vi "PicoScope6000aAWG.vi"(0 "Handle In":i16=16384, 1 "General AWG Settings":T4={"Peak-to-Peak Voltage"=2.0, "Offset Voltage"=0.0, "Wave Type"=17, "Sweep Type"=0, "Cycles"=10, "Trigger Type"=0, "Trigger Source"=4, "sigGenEnabled"=TRUE, "Trigger Enabled"=FALSE, "autoTriggerPicoSeconds"=0} {"Trigger Source" items=["None"=0, "Scope Trigger"=1, "Software Trigger"=4, "Trigger Raw"=5]; "Trigger Type" items=["Rising", "Falling", "Gate High", "Gate Low"]; "Sweep Type" items=["Up", "Down", "Up-Down", "Down-Up"]; "Wave Type" items=["Sine"=17, "Square"=18, "Triangle"=19, "Ramp Up"=20, "Ramp Down"=21, "Sinc"=22, "Gaussian"=23, "Half Sine"=24, "DC"=1024, "PWM"=4096, "White Noise"=8193, "PRBS"=8194, "Arbitrary"=268435456]; "Offset Voltage" format="%#_6p"; "Peak-to-Peak Voltage" format="%#_6p"}, 2 "Standard Waveform Settings":T3={"(Start) Frequency"=1000.0, "Stop Frequency"=5000.0, "Increment"=1.0, "Dwell Time (seconds)"=0.001, "Sweep Enabled"=FALSE} {"Dwell Time (seconds)" format="%#_6p"; "Stop Frequency" min=0.03 max=1000000.0 format="%#_6p"; "(Start) Frequency" min=0.03 max=1000000.0 format="%#_6p"}, 3 "Arbitrary Waveform Settings":T2 {"Index Mode" items=["Single", "Dual", "Quad"]}, 11 "error in":errorcluster, 12 "Duty Cycle":T1={"Use Duty Cycle"=FALSE, "dutyCyclePercent"=20.0}) -> (4 "Handle Out":i16=16384, 13 "Trigger Source Out":u32=4, 14 "Arbitrary\nWaveform Graph":i16[](graph), 15 "error out":errorcluster)   [LabVIEW 2010]
doc: "This VI can be used to control the arbitrary waveform generator. Standard waveforms can be selected or arbitrary waveform can be selected under 'Wave Type'. There are three settings clusters: general settings that apply to both arbitrary and standard waveforms, settings that apply only to standard waveforms and settings that apply only to arbitrary waveforms. It is not necessary to connect all of these clusters if only using arbitrary waveforms or only using standard waveforms are required.\n\nWhen selecting arbitrary waveform, it is necessary to specify a text file containing the wave form. This text file should have a single value on each line in the range -1 to 1. For further information on the settings, see descriptions of ps3000aSetSigGenBuiltIn and ps3000aSetSigGenArbitrary."
uses:
  ps6000a.dll
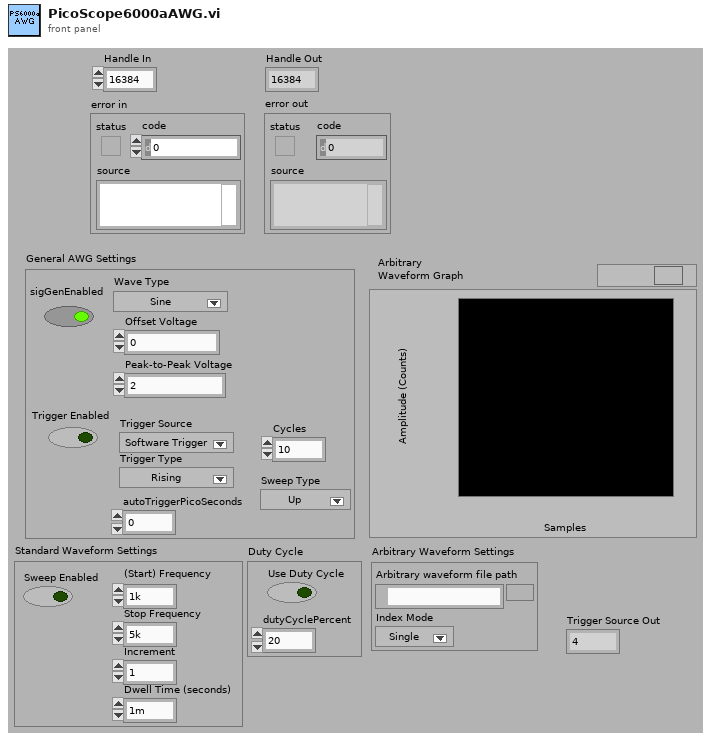
[diagram p1: front panel]
types:
  T1 = cluster{"Use Duty Cycle":bool, "dutyCyclePercent":dbl}
  T2 = cluster{"Arbirary waveform file path":path, "Index Mode":u32}
  T3 = cluster{"(Start) Frequency":dbl, "Stop Frequency":dbl, "Increment":dbl, "Dwell Time (seconds)":dbl, "Sweep Enabled":bool}
  T4 = cluster{"Peak-to-Peak Voltage":dbl, "Offset Voltage":dbl, "Wave Type":u32, "Sweep Type":u32, "Cycles":u64, "Trigger Type":u32, "Trigger Source":u32, "sigGenEnabled":bool, "Trigger Enabled":bool, "autoTriggerPicoSeconds":u64}
  T5 = cluster{"status":bool, "code":u32, "source":string}
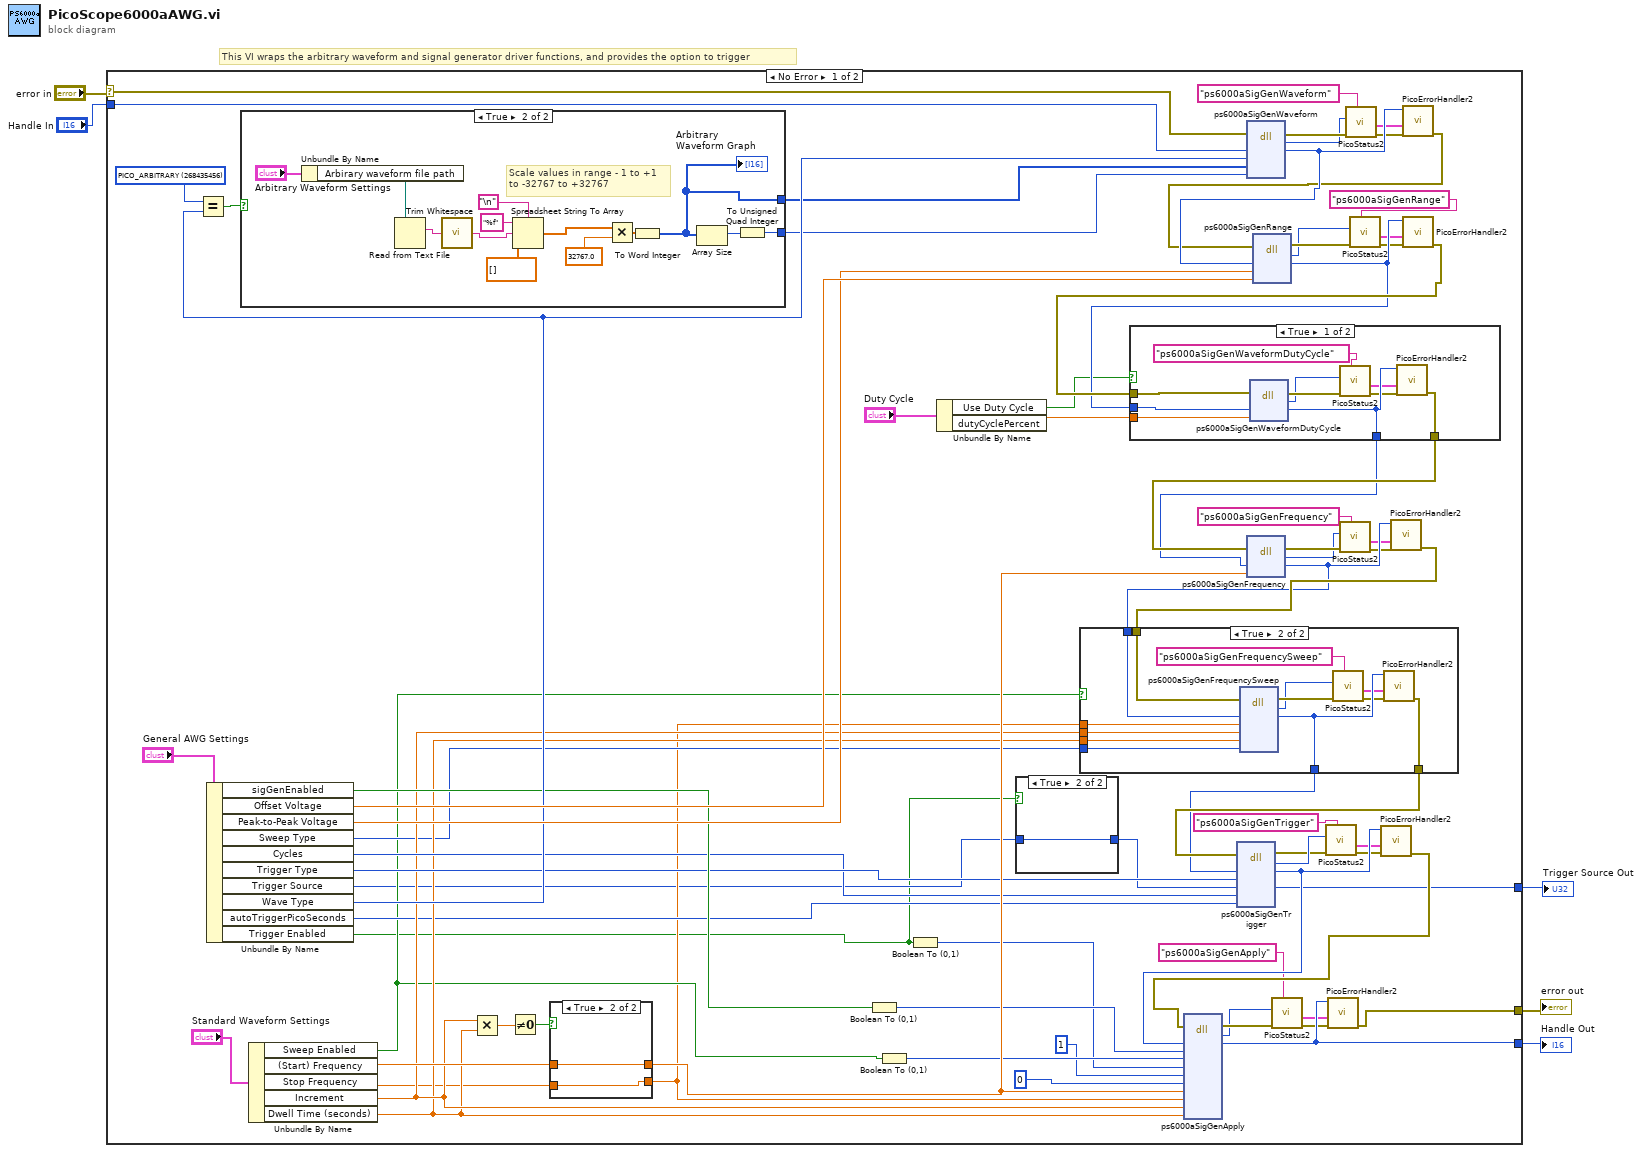
[diagram p0: block diagram]
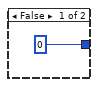
[diagram p2: hidden frame]
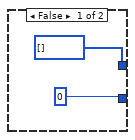
[diagram p4: hidden frame]
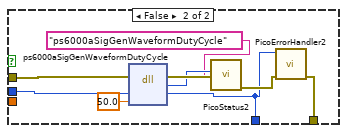
[diagram p5: hidden frame]
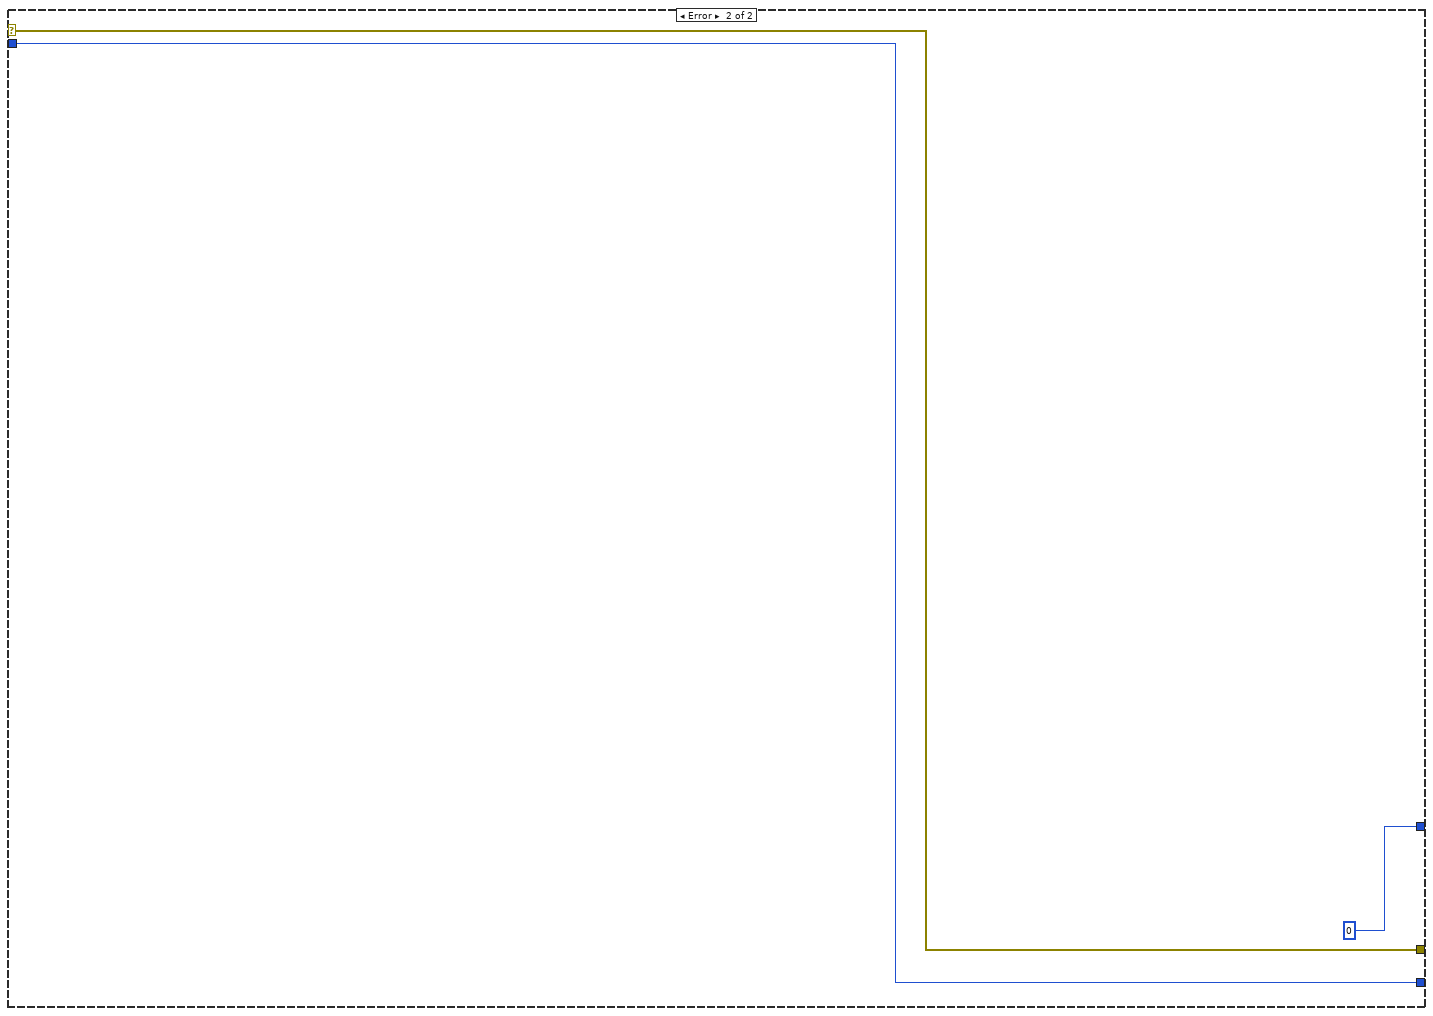
[diagram p7: hidden frame]
diagram:
  # "This VI wraps the arbitrary waveform and signal generator driver functions, and provides the option to trigger"
  n1 = case shown="No Error" "error in" {
    selector: "error in" -> [w76 w138]
    tunnel: [w70 w137] -> w5
    tunnel: "Handle In" -> [w81 w137]
    tunnel: [w69 w138] -> w3
    tunnel: [w34 0] -> w1
    frame No Error {
      w68 = u32 268435456 items=["PICO_ARBITRARY"=268435456]
      n2 = Unbundle By Name("General AWG Settings") -> ("sigGenEnabled"=w53:bool, "Offset Voltage"=w79:dbl, "Peak-to-Peak Voltage"=w78:dbl, "Sweep Type"=w38:u32, "Cycles"=w46:u64, "Trigger Type"=w47:u32, "Trigger Source"=w32:u32, "Wave Type"=w77:u32, "autoTriggerPicoSeconds"=w37:u64, "Trigger Enabled"=w31:bool)
      n3 = Equal?(x=w68, y=w77) -> (x = y?=w54:bool)
      n4 = case shown="True" w54 {
        tunnel: [i16[] [] ("buffer") w102] -> w61
        tunnel: [u64 0 ("bufferLenght") w101] -> w55
        frame False {
        }
        frame True {
          # "Scale values in range - 1 to +1 \nto -32767 to +32767"
          n5 = Unbundle By Name("Arbitrary Waveform Settings") -> ("Arbirary waveform file path"=w107:path)
          n6 = Read from Text File(file (use dialog)=w107) -> (text=w105:string)  [unwired: 3 in, 3 out]
          n7 = call <vilib>:"Trim Whitespace.vi"("string"=w105) -> ("trimmed string"=w104:string)  [unwired: 1 in]
          n8 = Spreadsheet String To Array(delimiter (Tab)="\n", format string="%f", spreadsheet string=w104, array type (2D Dbl)=dbl[] []) -> (array=w109:dbl[])
          n9 = Multiply(x=w109, y=32767.0 ("deltaPhaseIncrement")) -> (x*y=w106:dbl[])
          n10 = To Word Integer(number=w106) -> (16bit integer=w102:i16[])
          "Arbitrary\nWaveform Graph" <- w102
          n11 = Array Size(array=w102) -> (size(s)=w103:i32)
          n12 = To Unsigned Quad Integer(1:w103) -> (0:w101:u64)
        }
      }
      n13 = Unbundle By Name("Standard Waveform Settings") -> ("Sweep Enabled"=w36:bool, "(Start) Frequency"=w74:dbl, "Stop Frequency"=w43:dbl, "Increment"=w45:dbl, "Dwell Time (seconds)"=w44:dbl)
      n14 = Multiply(x=w45, y=w44) -> (x*y=w73:dbl)
      n15 = Not Equal To 0?(x=w73) -> (x != 0?=w72:bool)
      n16 = case shown="True" w72 {
        tunnel: [w133 w135] -> w35
        tunnel: w43 -> [_ w135]
        tunnel: w74 -> [w133 w134]
        tunnel: [w133 w134] -> w71
        frame False {
        }
        frame True {
        }
      }
      n17 = Boolean To (0,1)(Boolean=w53) -> (0, 1=w60:i16)
      n18 = Boolean To (0,1)(Boolean=w36) -> (0, 1=w59:i16)
      n19 = Boolean To (0,1)(Boolean=w31) -> (0, 1=w58:i16)
      n20 = Unbundle By Name("Duty Cycle") -> ("Use Duty Cycle"=w51:bool, "dutyCyclePercent"=w50:dbl)
      n21 = case shown="True" w31 {
        tunnel: [u32 0 ("Trigger Source") w83] -> w33
        tunnel: w32 -> [_ w83]
        frame False {
        }
        frame True {
        }
      }
      n22 = dll-call lib="ps6000a.dll" fn="ps6000aSigGenWaveform" ("ps3000.dll:_ps3000_open_unit@0")(error in=w76, "handle"=w81, "waveType"=w77, "buffer"=w61, "bufferLenght"=w55) -> (error out=w29:errorcluster, "PICO_STATUS"=w6:u32, "handle"=w67:i16)  [unwired: 5 in, 1 out]
      n23 = call "PicoStatus2.vi"("PICO source"="ps6000aSigGenWaveform" ("source"), "Error in"=w29, "PICO STATUS"=w6) -> ("error out"=w30:errorcluster, "PICO_STATUS out"=w26:T5)  [unwired: 5 in]
      n24 = call "PicoErrorHandler2.vi"("error in (no error)"=w30, "PICO_STATUS in"=w26, "handle In"=w67) -> ("error out"=w66:errorcluster)  [unwired: 8 in]
      n25 = dll-call lib="ps6000a.dll" fn="ps6000aSigGenRange" ("ps3000.dll:_ps3000_open_unit@0")(error in=w66, "handle"=w67, "peakToPeakVolts"=w78, "offsetVolts"=w79) -> (error out=w8:errorcluster, "PICO_STATUS"=w7:u32, "handle"=w64:i16)  [unwired: 4 in, 1 out]
      n26 = call "PicoStatus2.vi"("PICO source"="ps6000aSigGenRange" ("source"), "Error in"=w8, "PICO STATUS"=w7) -> ("error out"=w28:errorcluster, "PICO_STATUS out"=w25:T5)  [unwired: 5 in]
      n27 = call "PicoErrorHandler2.vi"("error in (no error)"=w28, "PICO_STATUS in"=w25, "handle In"=w64) -> ("error out"=w65:errorcluster)  [unwired: 8 in]
      n28 = case shown="True" w51 {
        tunnel: w65 -> [w123 w129]
        tunnel: w64 -> [w122 w128]
        tunnel: [w121 w127] -> w63
        tunnel: [w120 w126] -> w62
        tunnel: w50 -> [w119 _]
        frame True {
          n29 = dll-call lib="ps6000a.dll" fn="ps6000aSigGenWaveformDutyCycle" ("ps3000.dll:_ps3000_open_unit@0")(error in=w123, "handle"=w122, "dutyCyclePercent"=w119) -> (error out=w117:errorcluster, "PICO_STATUS"=w114:u32, "handle"=w120:i16)  [unwired: 3 in, 1 out]
          n30 = call "PicoStatus2.vi"("PICO source"="ps6000aSigGenWaveformDutyCycle" ("source"), "Error in"=w117, "PICO STATUS"=w114) -> ("error out"=w118:errorcluster, "PICO_STATUS out"=w116:T5)  [unwired: 5 in]
          n31 = call "PicoErrorHandler2.vi"("error in (no error)"=w118, "PICO_STATUS in"=w116, "handle In"=w120) -> ("error out"=w121:errorcluster)  [unwired: 8 in]
        }
        frame False {
          n32 = dll-call lib="ps6000a.dll" fn="ps6000aSigGenWaveformDutyCycle" ("ps3000.dll:_ps3000_open_unit@0")(error in=w129, "handle"=w128, "dutyCyclePercent"=50.0) -> (error out=w132:errorcluster, "PICO_STATUS"=w131:u32, "handle"=w126:i16)  [unwired: 3 in, 1 out]
          n33 = call "PicoStatus2.vi"("PICO source"="ps6000aSigGenWaveformDutyCycle" ("source"), "Error in"=w132, "PICO STATUS"=w131) -> ("error out"=w130:errorcluster)  [unwired: 5 in, 1 out]
          n34 = call "PicoErrorHandler2.vi"("error in (no error)"=w130, "handle In"=w126) -> ("error out"=w127:errorcluster)  [unwired: 9 in]
        }
      }
      n35 = dll-call lib="ps6000a.dll" fn="ps6000aSigGenFrequency" ("ps3000.dll:_ps3000_open_unit@0")(error in=w63, "handle"=w62, "frequencyHz"=w71) -> (error out=w10:errorcluster, "PICO_STATUS"=w9:u32, "handle"=w41:i16)  [unwired: 3 in, 1 out]
      n36 = call "PicoStatus2.vi"("PICO source"="ps6000aSigGenFrequency" ("source"), "Error in"=w10, "PICO STATUS"=w9) -> ("error out"=w27:errorcluster, "PICO_STATUS out"=w24:T5)  [unwired: 5 in]
      n37 = call "PicoErrorHandler2.vi"("error in (no error)"=w27, "PICO_STATUS in"=w24, "handle In"=w41) -> ("error out"=w42:errorcluster)  [unwired: 8 in]
      n38 = case shown="True" w36 {
        tunnel: w45 -> [_ w98]
        tunnel: w44 -> [_ w97]
        tunnel: w35 -> [_ w96]
        tunnel: w42 -> [w84 w95]
        tunnel: w41 -> [w85 w94]
        tunnel: [w84 w93] -> w40
        tunnel: [w85 w92] -> w39
        tunnel: w38 -> [_ w91]
        frame False {
        }
        frame True {
          n39 = dll-call lib="ps6000a.dll" fn="ps6000aSigGenFrequencySweep" ("ps3000.dll:_ps3000_open_unit@0")(error in=w95, "handle"=w94, "stopFrequencyHz"=w96, "frequencyIncrement"=w98, "dwellTimeSeconds"=w97, "sweepType"=w91) -> (error out=w87:errorcluster, "PICO_STATUS"=w86:u32, "handle"=w92:i16)  [unwired: 6 in, 1 out]
          n40 = call "PicoStatus2.vi"("PICO source"="ps6000aSigGenFrequencySweep" ("source"), "Error in"=w87, "PICO STATUS"=w86) -> ("error out"=w90:errorcluster, "PICO_STATUS out"=w89:T5)  [unwired: 5 in]
          n41 = call "PicoErrorHandler2.vi"("error in (no error)"=w90, "PICO_STATUS in"=w89, "handle In"=w92) -> ("error out"=w93:errorcluster)  [unwired: 8 in]
        }
      }
      n42 = dll-call lib="ps6000a.dll" fn="ps6000aSigGenTrigger" ("ps3000.dll:_ps3000_open_unit@0")(error in=w40, "handle"=w39, "triggerType"=w47, "triggerSource"=w33, "cycles"=w46, "autoTriggerPicoSeconds"=w37) -> (error out=w11:errorcluster, "PICO_STATUS"=w12:u32, "handle"=w48:i16, "triggerSource"=w34:u32)  [unwired: 5 in, 1 out]
      n43 = call "PicoStatus2.vi"("PICO source"="ps6000aSigGenTrigger" ("source"), "Error in"=w11, "PICO STATUS"=w12) -> ("error out"=w23:errorcluster, "PICO_STATUS out"=w22:T5)  [unwired: 5 in]
      n44 = call "PicoErrorHandler2.vi"("error in (no error)"=w23, "PICO_STATUS in"=w22, "handle In"=w48) -> ("error out"=w49:errorcluster)  [unwired: 8 in]
      n45 = dll-call lib="ps6000a.dll" fn="ps6000aSigGenApply" ("ps3000.dll:_ps3000_open_unit@0")(error in=w49, "handle"=w48, "sigGenEnabled"=w60, "sweepEnabled"=w59, "triggerEnabled"=w58, "automaticClockOptimisationEnabled"=i16 1, "overrideAutomaticClockAndPrescale"=i16 0, "frequency"=w71, "stopFrequency"=w35, "frequencyIncrement"=w45, "dwellTime"=w44) -> (error out=w14:errorcluster, "PICO_STATUS"=w13:u32, "handle"=w70:i16)  [unwired: 11 in, 1 out]
      n46 = call "PicoStatus2.vi"("PICO source"="ps6000aSigGenApply" ("source"), "Error in"=w14, "PICO STATUS"=w13) -> ("error out"=w21:errorcluster, "PICO_STATUS out"=w20:T5)  [unwired: 5 in]
      n47 = call "PicoErrorHandler2.vi"("error in (no error)"=w21, "PICO_STATUS in"=w20, "handle In"=w70) -> ("error out"=w69:errorcluster)  [unwired: 8 in]
    }
    frame Error {
    }
  }
  "Handle Out" <- w5
  "error out" <- w3
  "Trigger Source Out" <- w1
